vi "RemoteVI Status Registry.vi"(0 "publish?":bool, 1 "remove?":bool, 2 "status":T2) -> (4 "servers":T1(array[cluster]))   [LabVIEW 2020, in "RemoteVI.lvlib"]
doc: "Keeps the status of every RemoteVI share of this LabVIEW application instance - a functional global (a Feedback Node outside any loop, initialized on the first call only, so the list survives between calls of this non-reentrant VI). Each server loop publishes its entry every 500 ms (publish? TRUE, RemoteVI Publish Status.vi) - the entry of the same port is replaced, a new port is appended - and removes it when it stops (remove? TRUE, entry of status's port). Neither: servers is the list as it is (RemoteVI Status.vi, RemoteVI Start.vi). Times are seconds since the LabVIEW epoch (Get Date/Time In Seconds). An entry whose server loop was aborted stays, but stops being updated, so RemoteVI Status.vi reports it as stopped after 2 s. Pure G, no I/O."
uses:
  RemoteVI.lvlib
panel:
  in  "nothing yet":T1(array[cluster])
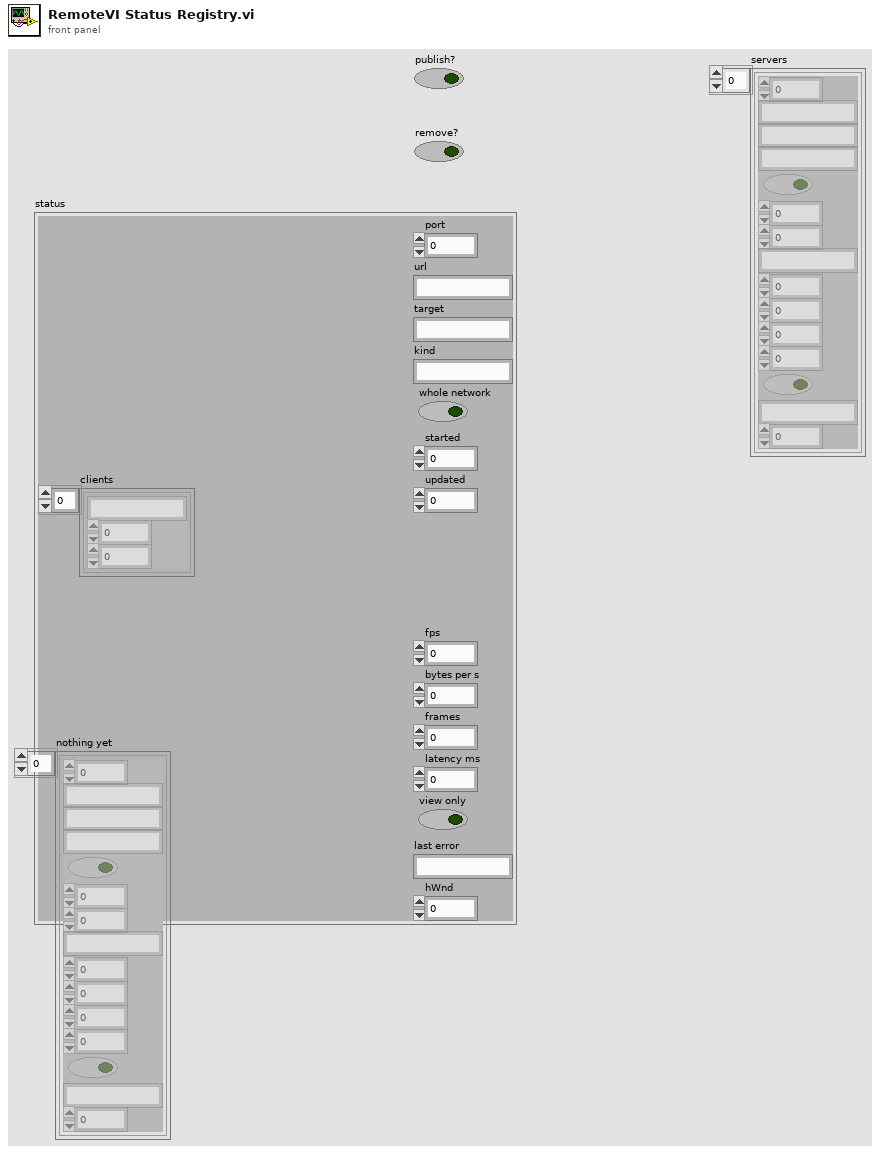
[diagram p1: front panel]
types:
  T1 = cluster{"port":u16, "url":string, "target":string, "kind":string, "whole network":bool, "started":dbl, "updated":dbl, "clients":cluster{"address":string, "since":dbl, "last input":dbl}[], "fps":dbl, "bytes per s":dbl, "frames":u32, "latency ms":dbl, "view only":bool, "last error":string, "hWnd":u64}[]
  T2 = cluster{"port":u16, "url":string, "target":string, "kind":string, "whole network":bool, "started":dbl, "updated":dbl, "clients":cluster{"address":string, "since":dbl, "last input":dbl}[], "fps":dbl, "bytes per s":dbl, "frames":u32, "latency ms":dbl, "view only":bool, "last error":string, "hWnd":u64}
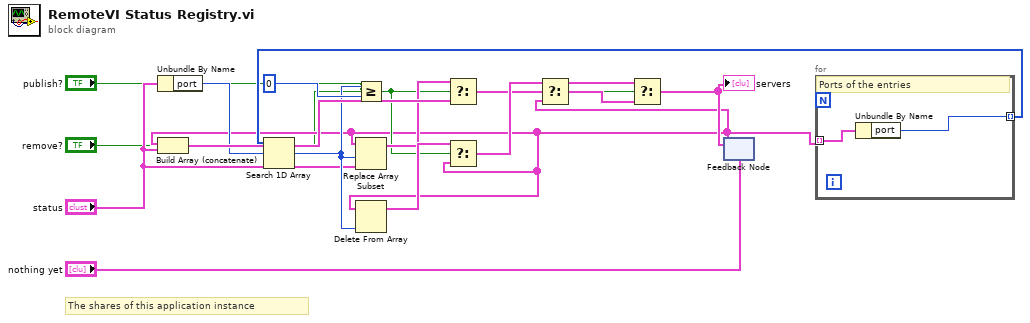
[diagram p0: block diagram]
diagram:
  # "The shares of this application instance"
  n1 = Unbundle By Name("status") -> ("port"=w7:u16)
  n2 = feedback #1("nothing yet") -> (w5:T1)
  n3 = Build Array (concatenate)(w5, "status") -> (w13:T1)
  n4 = for {
    tunnel: w5 -> [w18] mode=indexing
    tunnel: [w19] -> w8 mode=indexing
    # "Ports of the entries"
    n5 = Unbundle By Name(w18) -> ("port"=w19:u16)
  }
  n6 = Search 1D Array(1D array=w8, element=w7) -> (index of element=w9:i32)  [unwired: 1 in]
  n7 = Greater Or Equal?(x=w9, y=0) -> (x >= y?=w11:bool)
  n8 = Replace Array Subset(array=w5, new element="status", index=w9) -> (w12:T1)
  n9 = Delete From Array(array=w5, index=w9) -> (array with subset deleted=w15:T1)  [unwired: 1 in, 1 out]
  n10 = Select(t=w12, s=w11, f=w13) -> (s? t:f=w14:T1)
  n11 = Select(t=w15, s=w11, f=w5) -> (s? t:f=w16:T1)
  n12 = Select(t=w16, s="remove?", f=w5) -> (s? t:f=w17:T1)
  n13 = Select(t=w14, s="publish?", f=w17) -> (s? t:f=w6:T1)
  "servers" <- w6
  n14 = feedback-in #1(w6) -> ()
